vi "Update Value.vi"(6 "Time":dbl, 8 "error in (no error)":errorcluster, 11 "2WayValve in":refnum<class "2WayValveH.lvclass">) -> (0 "error out":errorcluster, 1 "Update":bool, 2 "Value":variant, 3 "2WayValve out":refnum<class "2WayValveH.lvclass">)   [LabVIEW 2020, in "VolatusGUIElements.lvlib" / "2WayValveH.lvclass"]
uses:
  2WayValveH.lvclass
  2WayValveH.lvclass/2WayValveH.ctl
  VolatusGUI/Element Inhibit/Element Inhibit.lvclass
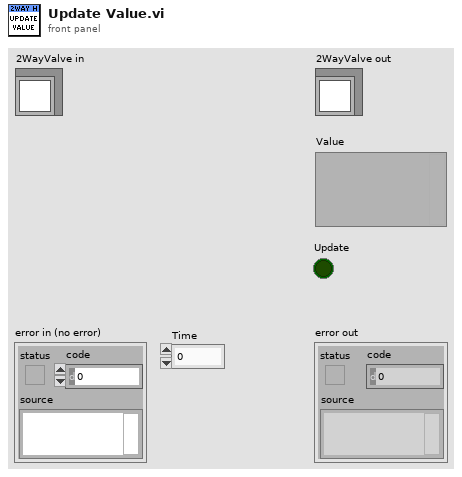
[diagram p1: front panel]
types:
  T1 = typedef "VolatusGUIElements.lvlib/2WayValveH.lvclass/Values.ctl" = cluster{"Command":T2, "CmdFB":T2, "Closed":T2, "Open":T2, "Energized":T2}
  T2 = typedef "VolatusGUIElements.lvlib/2WayValveH.lvclass/Channel State.ctl" = cluster{"Value":bool, "Stale":bool, "Config":bool, "Error":bool, "Prev":bool}
  T3 = typedef "VolatusGUIElements.lvlib/2WayValveH.lvclass/Unused Element.ctl" = cluster{"Command":bool, "Feedback":bool, "Energized":bool}
  T4 = typedef "VolatusGUIElements.lvlib/2WayValveH.lvclass/Picture.ctl" = enum16{"Blank", "OutClose", "OutOpen", "OutTranClose", "OutTranOpen", "OutConfig", "OutStale", "OutError", "InClose", "InOpen", "InTranClose", "InTranOpen", "InConfig", "InStale", "InError", "EnOff", "EnOn", "EnConfig", "EnStale", "EnError"}
  T5 = typedef "VolatusGUIElements.lvlib/2WayValveH.lvclass/Valve Pictures.ctl" = cluster{"Command":T6, "Feedback":T7, "Energized":T8}
  T6 = typedef "VolatusGUIElements.lvlib/2WayValveH.lvclass/Command Pictures.ctl" = cluster{"Error":T4, "Config":T4, "Stale":T4, "Close":T4, "Open":T4, "TranClose":T4, "TranOpen":T4}
  T7 = typedef "VolatusGUIElements.lvlib/2WayValveH.lvclass/Feedback Pictures.ctl" = cluster{"Error":T4, "Config":T4, "Stale":T4, "Closed":T4, "Open":T4, "TranClose":T4, "TranOpen":T4}
  T8 = typedef "VolatusGUIElements.lvlib/2WayValveH.lvclass/Energized Pictures.ctl" = cluster{"Error":T4, "Config":T4, "Stale":T4, "False":T4, "True":T4}
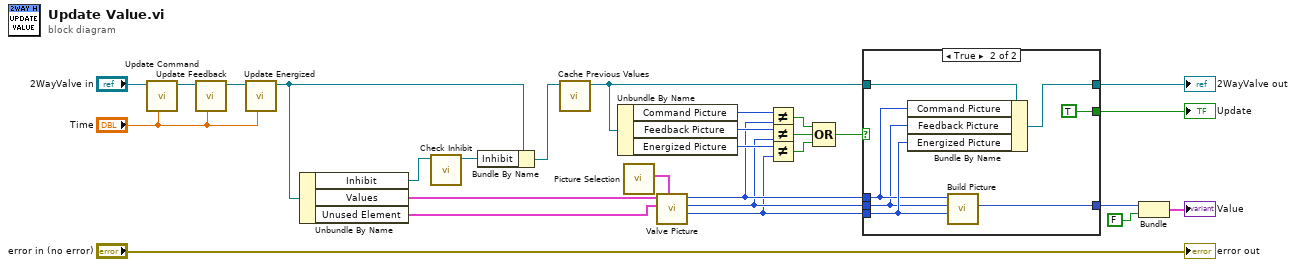
[diagram p0: block diagram]
diagram:
  n1 = call "Update Command.vi"("Time"="Time", "2WayValve in"="2WayValve in") -> ("2WayValve out"=w26:refnum<class "2WayValveH.lvclass">)  [unwired: 8 in, 1 out]
  n2 = call "Update Feedback.vi"("Time"="Time", "2WayValve in"=w26) -> ("2WayValve out"=w25:refnum<class "2WayValveH.lvclass">)  [unwired: 8 in, 1 out]
  n3 = call "Update Energized.vi"("Time"="Time", "2WayValve in"=w25) -> ("2WayValve out"=w4:refnum<class "2WayValveH.lvclass">)  [unwired: 8 in, 1 out]
  n4 = Unbundle By Name(w4) -> ("Inhibit"=w3:refnum<class "Element Inhibit.lvclass">, "Values"=w22:T1, "Unused Element"=w23:T3)
  n5 = call "Check Inhibit.vi"("Element Inhibit in"=w3) -> ("Element Inhibit out"=w1:refnum<class "Element Inhibit.lvclass">)  [unwired: 9 in, 1 out]
  n6 = Bundle By Name(cluster=w4, "Inhibit"=w1) -> (w2:refnum<class "2WayValveH.lvclass">)
  n7 = call "Cache Previous Values.vi"("2WayValve in"=w2) -> ("2WayValve out"=w7:refnum<class "2WayValveH.lvclass">)  [unwired: 9 in, 1 out]
  n8 = Unbundle By Name(w7) -> ("Command Picture"=w14:T4, "Feedback Picture"=w13:T4, "Energized Picture"=w12:T4)
  n9 = call "Picture Selection.vi"() -> ("Valve Pictures"=w20:T5)  [unwired: 11 in]
  n10 = call "Valve Picture.vi"("Valve Pictures"=w20, "Unused Element"=w23, "Values"=w22) -> ("Energized Picture"=w9:T4, "Feedback Picture"=w10:T4, "Command Picture"=w11:T4)  [unwired: 6 in]
  n11 = Not Equal?(x=w14, y=w11) -> (x != y?=w15:bool)
  n12 = Not Equal?(x=w13, y=w10) -> (x != y?=w17:bool)
  n13 = Not Equal?(x=w12, y=w9) -> (x != y?=w16:bool)
  n14 = Compound Arithmetic op=OR(w15, w17, w16) -> (w8:bool)
  n15 = case shown="True" w8 {
    tunnel: [_ w36] -> w18
    tunnel: w11 -> [_ w33]
    tunnel: w10 -> [_ w32]
    tunnel: w9 -> [_ w34]
    tunnel: w7 -> [w29 w35]
    tunnel: [w29 w31] -> w6
    tunnel: [_ TRUE] -> w5
    frame False {
    }
    frame True {
      n16 = Bundle By Name(cluster=w35, "Command Picture"=w33, "Feedback Picture"=w32, "Energized Picture"=w34) -> (w31:refnum<class "2WayValveH.lvclass">)
      n17 = call "Build Picture.vi"("Energized Picture"=w34, "Feedback Picture"=w32, "Command Picture"=w33) -> ("Valve Picture"=w36:picture)  [unwired: 8 in]
    }
  }
  "2WayValve out" <- w6
  "Update" <- w5
  n18 = Bundle("Valve Picture"=w18, FALSE) -> (→"Value":cluster{"Valve Picture":picture, bool})  [unwired: 1 in]
  "error out" <- "error in (no error)"
